vi "QueryFullProcessImageNameW Wrapper Template.vi"(0 "hProcess":u64, 5 "size":u32=1024, 7 "dwFlags":u32, 11 "error in":errorcluster) -> (4 "path":u16[](array[numeric]), 6 "return value":i32, 15 "error out":errorcluster)   [LabVIEW 2020]
doc: "Returns the full path of the program a process runs, as UTF-16 code units, through kernel32.dll QueryFullProcessImageNameW (stdcall, called in any thread). hProcess comes from kernel32 OpenProcess.vi with PROCESS_QUERY_LIMITED_INFORMATION. The buffer is size code units of zeros and the path is cut at its terminating 0. return value is the Win32 BOOL: non-zero on success. When error in carries an error the DLL is not called. Generated by tools\\Build Win32 Wrappers.vi - do not edit by hand, rebuild it."
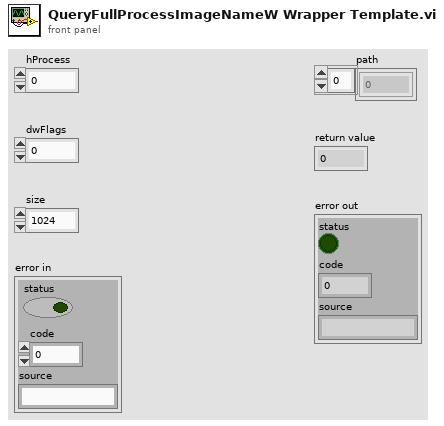
[diagram p1: front panel]
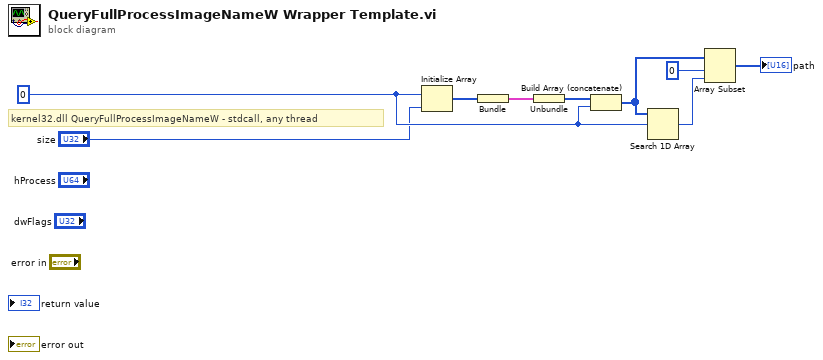
[diagram p0: block diagram]
diagram:
  w3 = u16 0
  # "kernel32.dll QueryFullProcessImageNameW - stdcall, any thread"
  n1 = Initialize Array(w3, "size") -> (w4:u16[])
  n2 = Bundle(w4) -> (w5:cluster{u16[]})  [unwired: 1 in]
  n3 = Unbundle(w5) -> (w6:u16[])
  n4 = Build Array (concatenate)(w6, w3) -> (w7:u16[])
  n5 = Search 1D Array(1D array=w7, element=w3) -> (index of element=w8:i32)  [unwired: 1 in]
  n6 = Array Subset(array=w7, index=0, length=w8) -> (→"path":u16[])
